vi "assets.get.vi"(8 "error in (no error)":errorcluster, 11 "Run in":refnum<class "Run.lvclass">) -> (0 "error out":errorcluster, 2 "Assets":refnum<class "asset.lvclass">[](array[class]), 3 "Run out":refnum<class "Run.lvclass">)   [LabVIEW 2020, in "Run.lvclass"]
uses:
  Run.lvclass
  Run.lvclass/Run.ctl
  fc990382-c15b-405e-8523-435b97eca7cf.vi
  fc990382-c15b-405e-8523-435b97eca7cf.vi/32c3acc2-0975-485a-8283-62feb0f3dc4f.vi
  run_properties.get.vi
  <vilib>/JDP Science/JSONtext/JSON type.vi
  <vilib>/JDP Science/JSONtext/JSON text to Variant.vi
  <vilib>/JDP Science/JSONtext/LVClass Serializer/JSONtext LVClass Serializer.lvclass
  Nominal Client/Nominal Client.lvclass
  asset/asset.lvclass
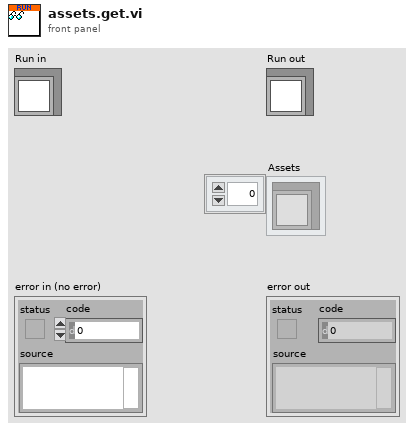
[diagram p1: front panel]
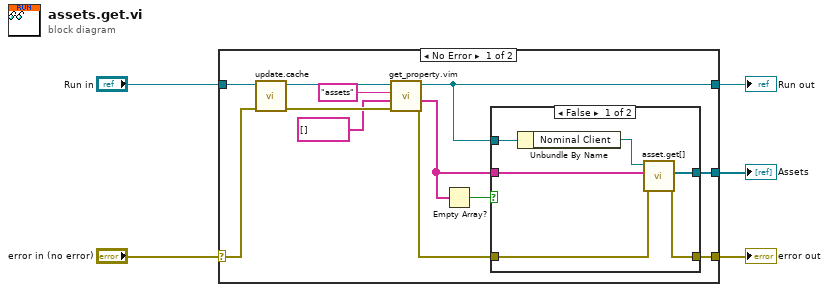
[diagram p0: block diagram]
diagram:
  n1 = case shown="No Error" "error in (no error)" {
    selector: "error in (no error)" -> [w17 w25]
    tunnel: [w9 w25] -> w4
    tunnel: [w8 w26] -> w2
    tunnel: "Run in" -> [w16 w26]
    tunnel: [w11 _] -> w1
    frame No Error {
      n2 = call "update.cache.vi"("error in"=w17, "Run in"=w16) -> ("error out"=w14:errorcluster, "Run out"=w15:refnum<class "Run.lvclass">)  [unwired: 8 in]
      n3 = call "get_property.vim"("error in"=w14, "default value and type"=string[] [] ("assets"), "Property Name"="assets", "Run in"=w15) -> ("error out"=w10:errorcluster, "Value"=w7:string[], "Run out"=w8:refnum<class "Run.lvclass">)  [unwired: 5 in]
      n4 = Empty Array?(array=w7) -> (empty?=w6:bool)
      n5 = case shown="False" w6 {
        tunnel: [w23 _] -> w11
        tunnel: w10 -> [w22 w24]
        tunnel: [w21 w24] -> w9
        tunnel: w8 -> [w20 _]
        tunnel: w7 -> [w18 _]
        frame False {
          n6 = Unbundle By Name(w20) -> ("Nominal Client"=w19:refnum<class "Nominal Client.lvclass">)
          n7 = call "asset.get[].vi"("error in"=w22, "Asset RIDs"=w18, "Nominal Client in"=w19) -> ("error out"=w21:errorcluster, "Assets"=w23:refnum<class "asset.lvclass">[])  [unwired: 6 in, 1 out]
        }
        frame True {
        }
      }
    }
    frame Error {
    }
  }
  "error out" <- w4
  "Run out" <- w2
  "Assets" <- w1
